vi "GetRingText.vi"(8 "error in (no error)":errorcluster, 11 "RingItem in":refnum<class "RingItem.lvclass">) -> (0 "error out":errorcluster, 2 "ring text":string, 3 "RingItem out":refnum<class "RingItem.lvclass">)   [LabVIEW 2023, in "GettingStartedWindow.lvlib" / "RingItem.lvclass"]
uses:
  <resource>/modes/FRC/GSW/Classes/RingItem/RingItem.lvclass
  <resource>/modes/FRC/GSW/Classes/RingItem/RingItem.lvclass/RingItem.ctl
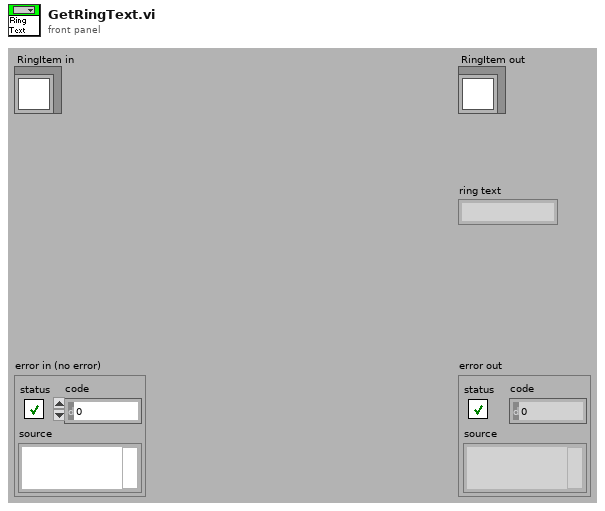
[diagram p1: front panel]
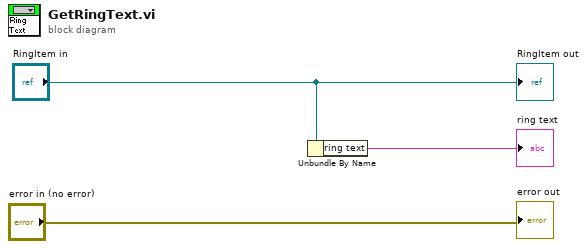
[diagram p0: block diagram]
diagram:
  n1 = Unbundle By Name("RingItem in") -> ("ring text"=→"ring text":string)
  "error out" <- "error in (no error)"
  "RingItem out" <- "RingItem in"
